vi "DAC Configure.vi"(8 "error in":errorcluster, 11 "DAC HeatFlow AIV in":refnum<class "DAC HeatFlow AIV.lvclass">) -> (0 "error out":errorcluster, 3 "DAC HeatFlow AIV out":refnum<class "DAC HeatFlow AIV.lvclass">)   [LabVIEW 2019, in "DAC.lvlib" / "DAC HeatFlow AIV.lvclass"]
uses:
  DAC HeatFlow AIV.lvclass
  C:/Users/krio/Documents/LV_Projects/test-stand/App/DAC/DAC.lvclass
  DAC.lvclass/DAC.ctl
  DAC HeatFlow AIV.lvclass/DAC HeatFlow AIV.ctl
  <vilib>/Utility/error.llb/Error Cluster From Error Code.vi
  <vilib>/DAQmx/create/channels.llb/DAQmx Create Channel (AI-Voltage-Basic).vi
  <vilib>/ErrorRing/Error Ring.xnode
  DAC.lvclass
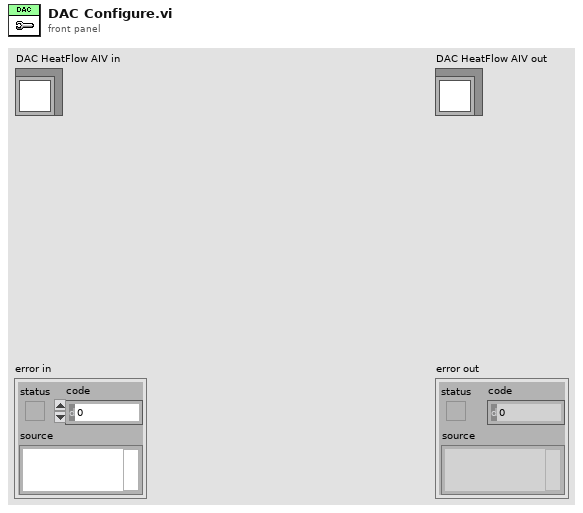
[diagram p1: front panel]
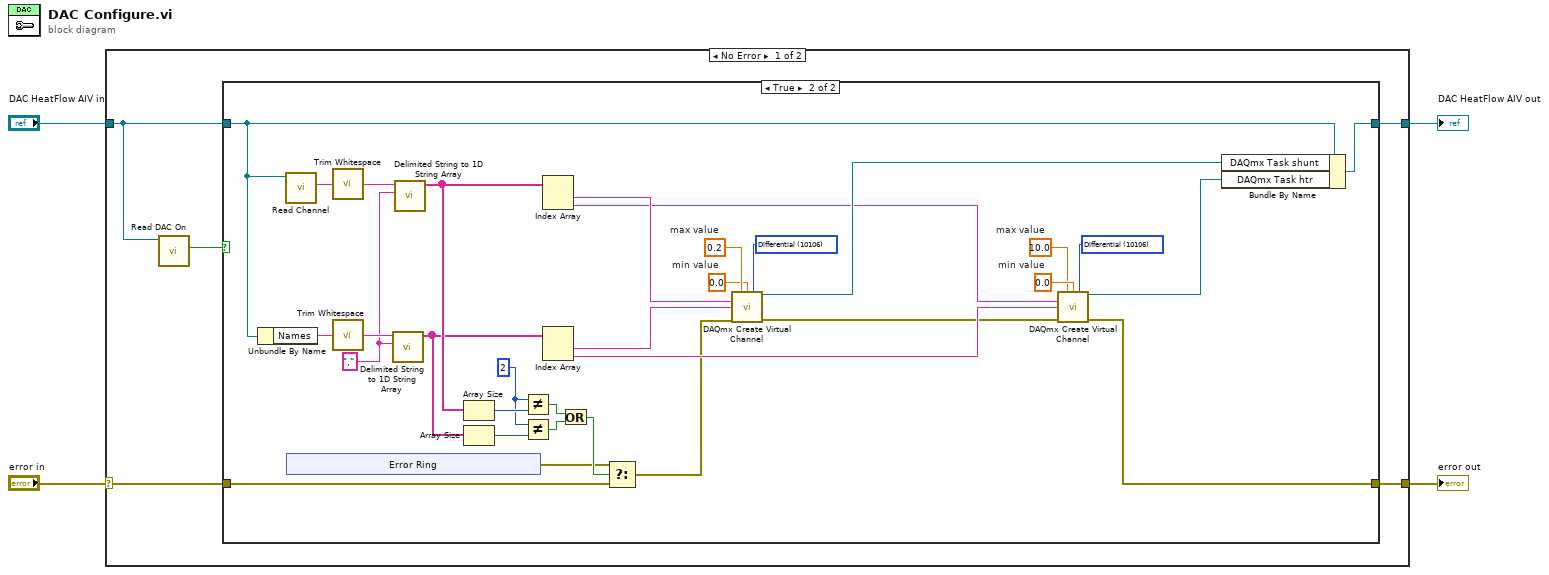
[diagram p0: block diagram]
diagram:
  n1 = case shown="No Error" "error in" {
    selector: "error in" -> [w6 w49]
    tunnel: [w5 w49] -> w4
    tunnel: [w7 w48] -> w3
    tunnel: "DAC HeatFlow AIV in" -> [w9 w48]
    frame No Error {
      n2 = call "Read DAC On.vi"("DAC in"=w9) -> ("DAC On"=w8:bool)  [unwired: 8 in, 2 out]
      n3 = case shown="True" w8 {
        tunnel: w9 -> [w11 w42]
        tunnel: [w11 w43] -> w7
        tunnel: w6 -> [w10 w26]
        tunnel: [w10 w17] -> w5
        frame False {
        }
        frame True {
          w20 = 10106 items=["Default"=-1, "RSE"=10083, "NRSE"=10078, "Differential"=10106, "Pseudodifferential"=12529] ("input terminal configuration")
          w19 = 0.0  # min value
          w18 = 10.0  # max value
          w30 = 2 ("x")
          w33 = "," ("delimiter")
          w38 = 10106 items=["Default"=-1, "RSE"=10083, "NRSE"=10078, "Differential"=10106, "Pseudodifferential"=12529] ("input terminal configuration")
          w39 = 0.0  # min value
          w40 = 0.2  # max value
          n4 = Unbundle By Name(w42) -> ("Names"=w36:string)
          n5 = call "Read Channel.vi"("DAC in"=w42) -> ("Channel"=w37:string)  [unwired: 8 in, 2 out]
          n6 = xnode "Error Ring"() -> ("error out"=w25:errorcluster)
          n7 = call <vilib>:"Trim Whitespace.vi"("string"=w37) -> ("trimmed string"=w35:string)  [unwired: 1 in]
          n8 = call <vilib>:"Trim Whitespace.vi"("string"=w36) -> ("trimmed string"=w34:string)  [unwired: 1 in]
          n9 = call <vilib>:"Delimited String to 1D String Array.vi"("delimiter"=w33, "delimited string"=w34) -> ("string array"=w23:string[])  [unwired: 9 in]
          n10 = call <vilib>:"Delimited String to 1D String Array.vi"("delimiter"=w33, "delimited string"=w35) -> ("string array"=w24:string[])  [unwired: 9 in]
          n11 = Array Size(array=w24) -> (size(s)=w32:i32)
          n12 = Array Size(array=w23) -> (size(s)=w31:i32)
          n13 = Not Equal?(x=w30, y=w32) -> (x != y?=w29:bool)
          n14 = Not Equal?(x=w30, y=w31) -> (x != y?=w28:bool)
          n15 = Index Array(array=w24) -> (element #1=w22:string, element #2=w15:string)  [unwired: 2 in]
          n16 = Index Array(array=w23) -> (element #1=w21:string, element #2=w14:string)  [unwired: 2 in]
          n17 = Or(x=w29, y=w28) -> (x .or. y?=w27:bool)
          n18 = Select(t=w25, s=w27, f=w26) -> (s? t:f=w13:errorcluster)
          n19 = call-poly <vilib>:"DAQmx Create Virtual Channel.vi"("maximum value"=w40, "minimum value"=w39, "input terminal configuration"=w38, "physical channels"=w22, "name to assign"=w21, "error in"=w13) -> ("task out"=w41:refnum<k21>, "error out"=w12:errorcluster)  [unwired: 8 in]
          n20 = call-poly <vilib>:"DAQmx Create Virtual Channel.vi"("maximum value"=w18, "minimum value"=w19, "input terminal configuration"=w20, "physical channels"=w15, "name to assign"=w14, "error in"=w12) -> ("task out"=w16:refnum<k21>, "error out"=w17:errorcluster)  [unwired: 8 in]
          n21 = Bundle By Name(cluster=w42, "DAQmx Task shunt"=w41, "DAQmx Task htr"=w16) -> (w43:refnum<class "DAC HeatFlow AIV.lvclass">)
        }
      }
    }
    frame Error {
    }
  }
  "error out" <- w4
  "DAC HeatFlow AIV out" <- w3
